vi "create asset.vi"(9 "Description":string, 10 "Title":string, 11 "connection":refnum<class "Nominal Client.lvclass">) -> (0 "error out":errorcluster, 3 "asset":refnum<class "asset.lvclass">)   [LabVIEW 2020, in "nominal core steps.lvlib"]
doc: "Creates a new metadata asset in Nominal.\n<b> </b> <b> </b>"
uses:
  nominal core steps.lvlib
  <vilib>/Nominal/Nominal IO Client/lv_src/Nominal Client/Nominal Client.lvclass
  <vilib>/Nominal/Nominal IO Client/lv_src/asset/asset.lvclass
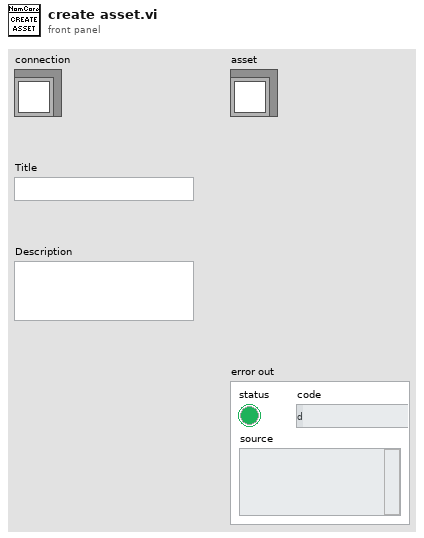
[diagram p1: front panel]
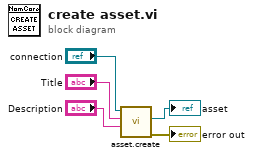
[diagram p0: block diagram]
diagram:
  n1 = call <vilib>:"asset.create.vi"("Description"="Description", "Title"="Title", "Nominal Client in"="connection") -> ("error out"=→"error out":errorcluster, "asset"=→"asset":refnum<class "asset.lvclass">)  [unwired: 6 in, 1 out]
